vi "LabVIEW.Service.Timer.vi"(0 "Loop Iteration":i32, 1 "Loop Timeout (10s)":u32=10, 6 "User Condition":bool, 8 "Error In (no error)":errorcluster) -> (7 "Timeout?":bool, 10 "Error Out":errorcluster)   [LabVIEW 2019]
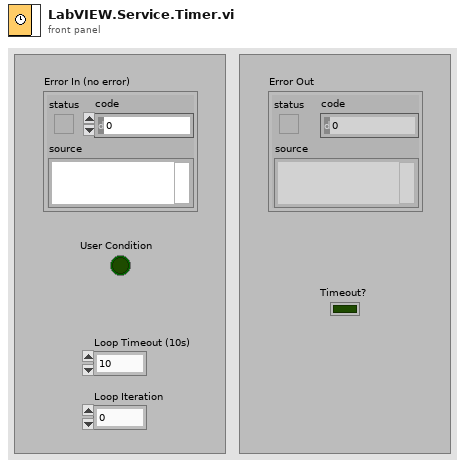
[diagram p1: front panel]
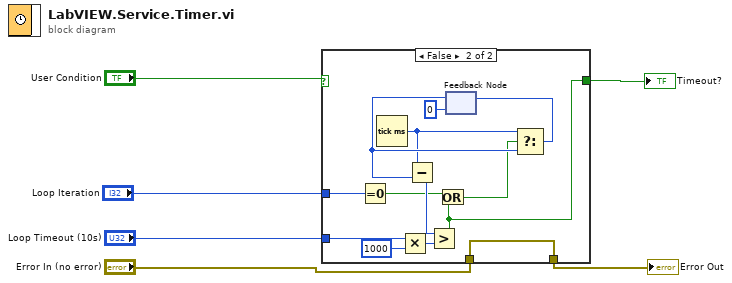
[diagram p0: block diagram]
diagram:
  n1 = case shown="False" "User Condition" {
    selector: "User Condition" -> [w8 _]
    tunnel: "Loop Iteration" -> [_ w21]
    tunnel: "Loop Timeout (10s)" -> [_ w18]
    tunnel: [w8 w9] -> w3
    tunnel: "Error In (no error)" -> [w7 w10]
    tunnel: [w7 w10] -> w1
    frame True {
    }
    frame False {
      n2 = Equal To 0?(x=w21) -> (x = 0?=w12:bool)
      n3 = Tick Count (ms)() -> (millisecond timer value=w16:u32)
      n4 = Multiply(x=w18, y=u32 1000) -> (x*y=w17:u32)
      n5 = feedback #1(u32 0 ("millisecond timer value")) -> (w20:u32)
      n6 = Subtract(x=w16, y=w20) -> (x-y=w13:u32)
      n7 = Greater?(x=w13, y=w17) -> (0:w9:bool)
      n8 = Or(x=w12, y=w9) -> (x .or. y?=w11:bool)
      n9 = Select(t=w16, s=w11, f=w20) -> (s? t:f=w14:u32)
      n10 = feedback-in #1(w14) -> ()
    }
  }
  "Error Out" <- w1
  "Timeout?" <- w3
